vi "Symulacja_pomiaru.vi"(1 "poprzednia_dana":dbl) -> (0 "Biezaca_dana":dbl)   [LabVIEW 2026]
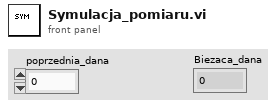
[diagram p1: front panel]
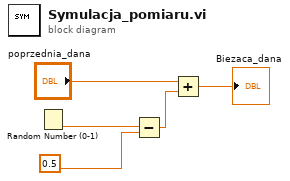
[diagram p0: block diagram]
diagram:
  n1 = Random Number (0-1)() -> (number: 0 to 1=w2:dbl)
  n2 = Subtract(x=w2, y=0.5) -> (x-y=w1:dbl)
  n3 = Add(x="poprzednia_dana", y=w1) -> (x+y=→"Biezaca_dana":dbl)
